vi "VIH HelpGen - Get Target Folder for an Output File.vi"(9 "Item/File Type":T1, 10 "File Path":path, 11 "Target Paths":T2) -> (3 "Target Folder":path)   [LabVIEW 2014]
doc: "::: VI Helpeks :::\nCopyright (c) 2000-2026 Konstantin Shifershteyn. All rights reserved."
uses:
  VIH HelpGen Typedef - Cluster - File Rule - Target Paths.ctl
  _VIH HelpGen - Palette.llb/VIH HelpGen Typedef - Palette - Item Type Enum.ctl
panel:
  # "VI Helpeks\nCopyright (c) 2012-2026 Konstantin Shifershteyn"
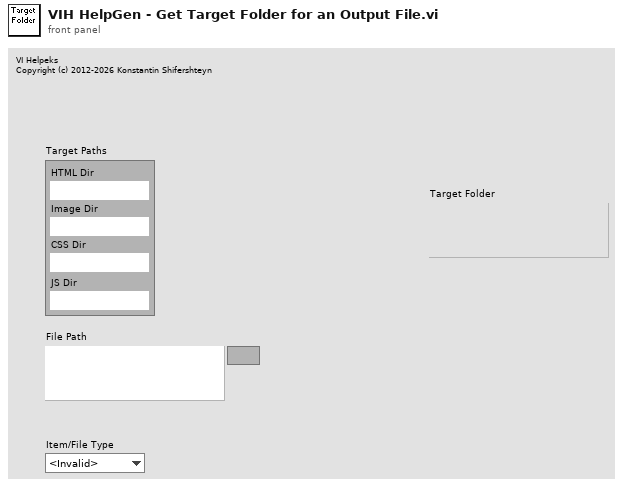
[diagram p1: front panel]
types:
  T1 = typedef "VIH HelpGen Typedef - Palette - Item Type Enum.ctl" = enum32{"<Invalid>", "<unknown>", "VI", "Menu", "LV Func", "Express VI", "Poly VI", "CTL", "HTML"}
  T2 = typedef "VIH HelpGen Typedef - Cluster - File Rule - Target Paths.ctl" = cluster{"HTML Dir":path, "Image Dir":path, "CSS Dir":path, "JS Dir":path}
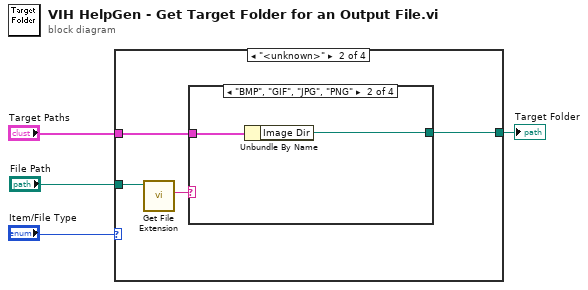
[diagram p0: block diagram]
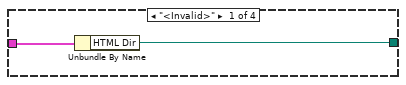
[diagram p2: hidden frame]
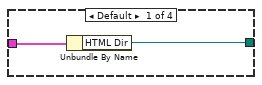
[diagram p3: hidden frame]
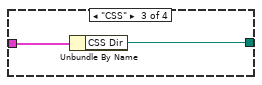
[diagram p4: hidden frame]
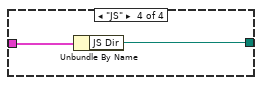
[diagram p5: hidden frame]
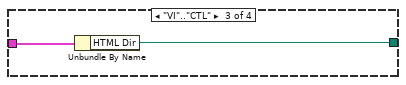
[diagram p6: hidden frame]
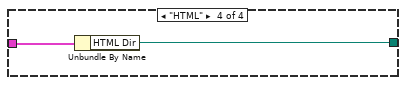
[diagram p7: hidden frame]
diagram:
  n1 = case shown="\"<unknown>\"" "Item/File Type" {
    tunnel: "File Path" -> [_ w9 _ _]
    tunnel: [w5 w8 w19 w21] -> w3
    tunnel: "Target Paths" -> [w6 w7 w20 w22]
    frame "<Invalid>" {
      n2 = Unbundle By Name(w6) -> ("HTML Dir"=w5:path)
    }
    frame "<unknown>" {
      n3 = call <vilib>:"Get File Extension.vi"("file"=w9) -> ("lowercase file extension"=w10:string)  [unwired: 7 in, 3 out]
      n4 = case shown="\"BMP\", \"GIF\", \"JPG\", \"PNG\"" w10 {
        tunnel: w7 -> [w12 w14 w16 w18]
        tunnel: [w11 w13 w15 w17] -> w8
        frame Default {
          n5 = Unbundle By Name(w12) -> ("HTML Dir"=w11:path)
        }
        frame "BMP", "GIF", "JPG", "PNG" {
          n6 = Unbundle By Name(w14) -> ("Image Dir"=w13:path)
        }
        frame "CSS" {
          n7 = Unbundle By Name(w16) -> ("CSS Dir"=w15:path)
        }
        frame "JS" {
          n8 = Unbundle By Name(w18) -> ("JS Dir"=w17:path)
        }
      }
    }
    frame "VI".."CTL" {
      n9 = Unbundle By Name(w20) -> ("HTML Dir"=w19:path)
    }
    frame "HTML" {
      n10 = Unbundle By Name(w22) -> ("HTML Dir"=w21:path)
    }
  }
  "Target Folder" <- w3
